vi "build.epoch.vi"(10 "Time Unit":T1(ring), 11 "Time Series Name":string) -> (3 "Timestamp Metadata":refnum<class "timestampMetadata.lvclass">)   [LabVIEW 2020, in "ts.epochOfTimeUnit.lvclass"]
uses:
  ts.epochOfTimeUnit.lvclass
  ts.epochOfTimeUnit.lvclass/ts.epochOfTimeUnit.ctl
  timestampMetadata/timestampMetadata.lvclass
  C:/code/labview-client/lv_src/ts.absoloute type/ts.absoloute type.lvclass
  C:/code/labview-client/lv_src/timestampType/timestampType.lvclass
  C:/code/labview-client/lv_src/Nominal Client/datasources/payload/payload.lvclass
  C:/code/labview-client/lv_src/ts.epochOfTimeUnit/ts.epochOfTimeUnit.lvclass
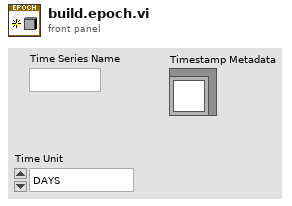
[diagram p1: front panel]
types:
  T1 = enum16{"DAYS", "HOURS", "MINUTES", "SECONDS", "MILLISECONDS", "MICROSECONDS", "NANOSECONDS", "PICOSECONDS"}
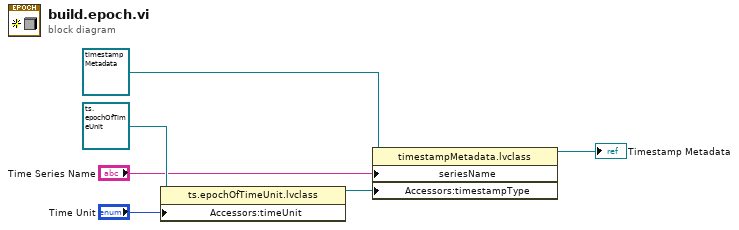
[diagram p0: block diagram]
diagram:
  n1 = property class="ts.epochOfTimeUnit.lvclass"(reference=refnum<class "ts.epochOfTimeUnit.lvclass"> refnum ("ts.epochOfTimeUnit in"), "Accessors:timeUnit"="Time Unit") -> (reference out=w2:refnum<class "ts.epochOfTimeUnit.lvclass">)  [unwired: 1 in, 1 out]
  n2 = property class="timestampMetadata.lvclass"(reference=refnum<class "timestampMetadata.lvclass"> refnum ("Timestamp Metadata"), "seriesName"="Time Series Name", "Accessors:timestampType"=w2) -> (reference out=→"Timestamp Metadata":refnum<class "timestampMetadata.lvclass">)  [unwired: 1 in, 1 out]
